vi "Measurement UI.vi"() -> ()   [LabVIEW 2022 SP3, in "Generation_Class D Amplifier_UI.lvlib"]
uses:
  Generation_Class D Amplifier_UI.lvlib
  Generation_Class D Amplifier/generation control.ctl
  shared/controls/digital output level units.ctl
  service/generation/controls/generation status.ctl
  shared/controls/generation type.ctl
  state.ctl
  <vilib>/Utility/miscctls.llb/LVPositionTypeDef.ctl
  <vilib>/Utility/miscctls.llb/LVRowAndColumnTypeDef.ctl
  service/generation/API/AudioGeneration/AudioGeneration.lvclass
  service/generation/controls/generation type.ctl
  service/generation/controls/AudioGenTypeDefs.lvlib
  shared/audio popup ui/Audio Popup UI.lvlib
  shared/controls/audio controls.lvlib
  Generation_Class D Amplifier/Generation_Class D Amplifier.lvlib
  shared/digital serial gen settings/digital audio protocol controls.lvlib
panel:
  out "placeholder":string
  in  "signal parameters":string
  in  "sine wave table":string[][](table)
  in  "DAQmx Physical Channel":tag caption="Analog output channel"
  in  "configure output":bool
  in  "output type":T1 caption="Generation Type"
  in  "master clock channel list":string caption="Master clock channel"
  in  "digital channel list":string caption="Digital audio channel"
  in  "analog output channel":string
  in  "output configuration file":string
  out "status":T2 caption="Status"
  in  "output level units":T3 caption="Output level units"
  in  "generation control":T4=enum."Stop" caption="Action"
  # "Generation"
  # "Harware Resource"
  # "Signals"
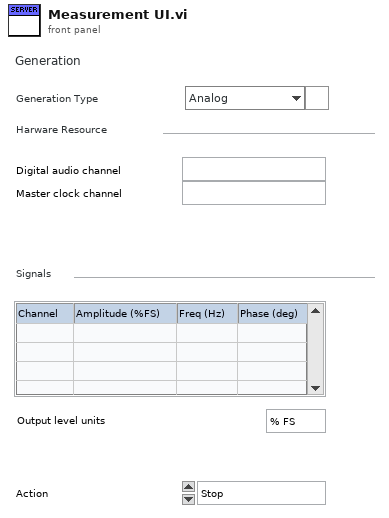
[diagram p1: front panel]
types:
  T1 = typedef "generation type.ctl" = enum32{"Analog", "Digital Serial"}
  T2 = typedef "AudioGenTypeDefs.lvlib/generation status.ctl" = enum16{"Idle", "Committed", "Active"}
  T3 = typedef "audio controls.lvlib/digital output level units.ctl" = enum32{"% FS", "dBFS", "V"}
  T4 = typedef "Generation_Class D Amplifier.lvlib/generation control.ctl" = enum32{"Start", "Stop"}
  T5 = typedef "Generation_Class D Amplifier_UI.lvlib/state.ctl" = cluster{"PostUI event occurred":bool, "digital serial cfg file":path, "analog cfg file":path, "number of channels":u32}
  T6 = typedef "LVPositionTypeDef.ctl" = cluster{"Left":i32, "Top":i32}
  T7 = typedef "LVRowAndColumnTypeDef.ctl" = cluster{"Row":i32, "Column":i32}
  T8 = typedef "AudioGenTypeDefs.lvlib/generation type.ctl" = enum16{"analog", "digital"}
  T9 = cluster{"frequency":dbl, "amplitude":dbl, "phase":dbl}[]
  T10 = typedef "digital serial gen settings.ctl" = cluster{"number of channels":u32, "data justification":T11, "endianness":T12, "channel length":u32, "bit depth":u32, "frame clock rate":dbl, "bit clock edge sync":T13, "master clock rate":dbl, "Logic Level":T14, "frame sync edge for channel 0":T13, "Channel 0 Offset":u32}
  T11 = typedef "PDM Shared.lvlib/PCM Data Justification.ctl" = enum16{"Left Justified", "Right Justified"}
  T12 = typedef "PDM Shared.lvlib/PCM Bit Endianness.ctl" = enum16{"MSB First", "LSB First"}
  T13 = typedef "PDM Shared.lvlib/Digital Edge.ctl" = enum8{"Rising", "Falling"}
  T14 = typedef "PDM Acquisition Class Library.lvlib/DecoderSession.lvclass/Logic Levels.ctl" = enum16{"3.3 V", "1.8 V", "1.2 V"}
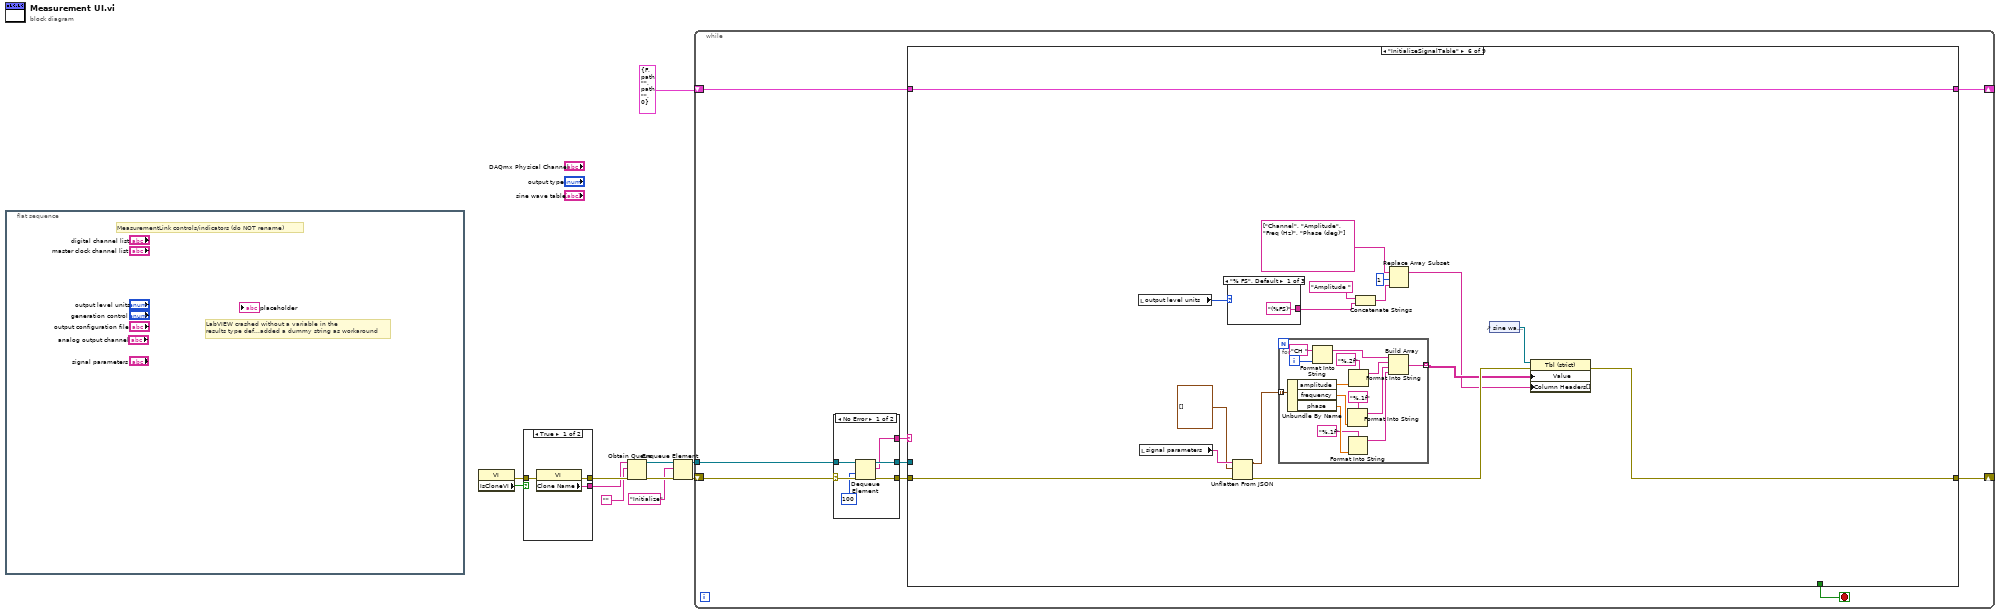
[diagram p0: block diagram]
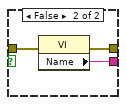
[diagram p2: hidden frame]
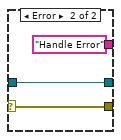
[diagram p3: hidden frame]
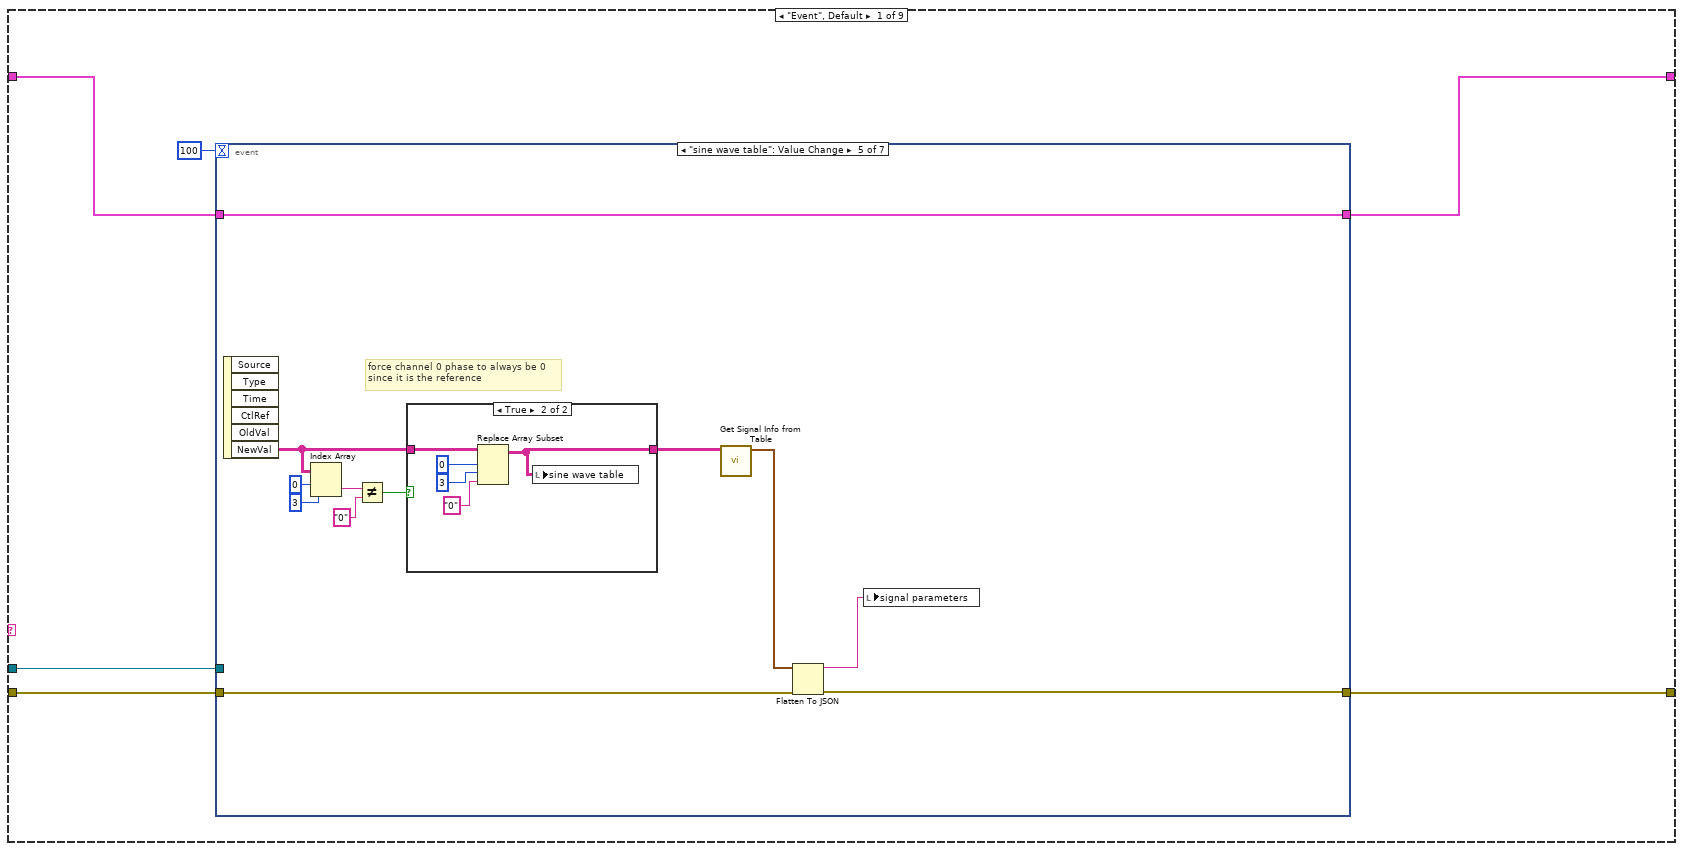
[diagram p4: hidden frame]
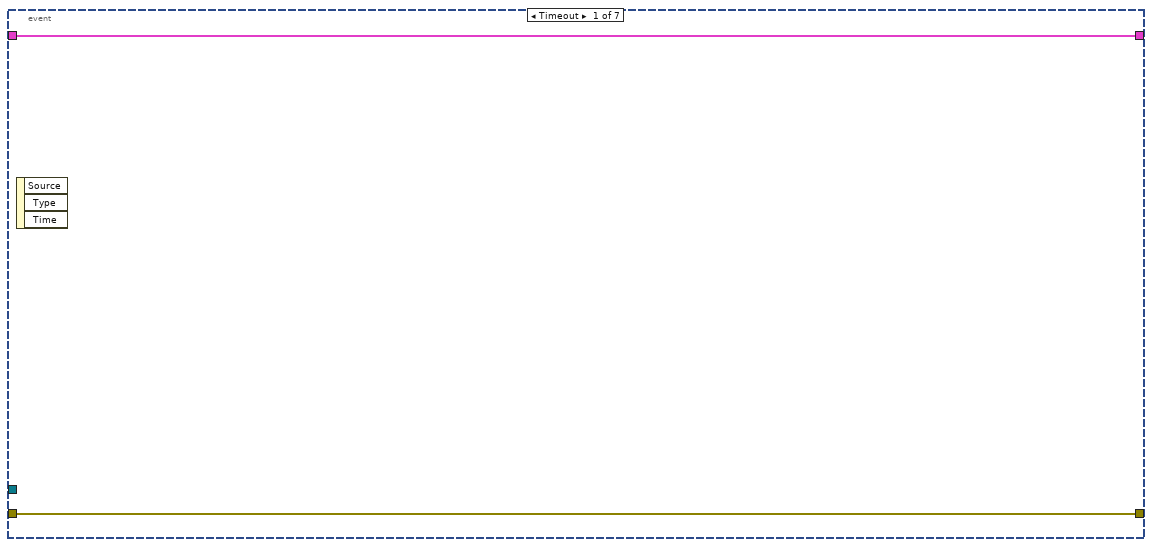
[diagram p5: hidden frame]
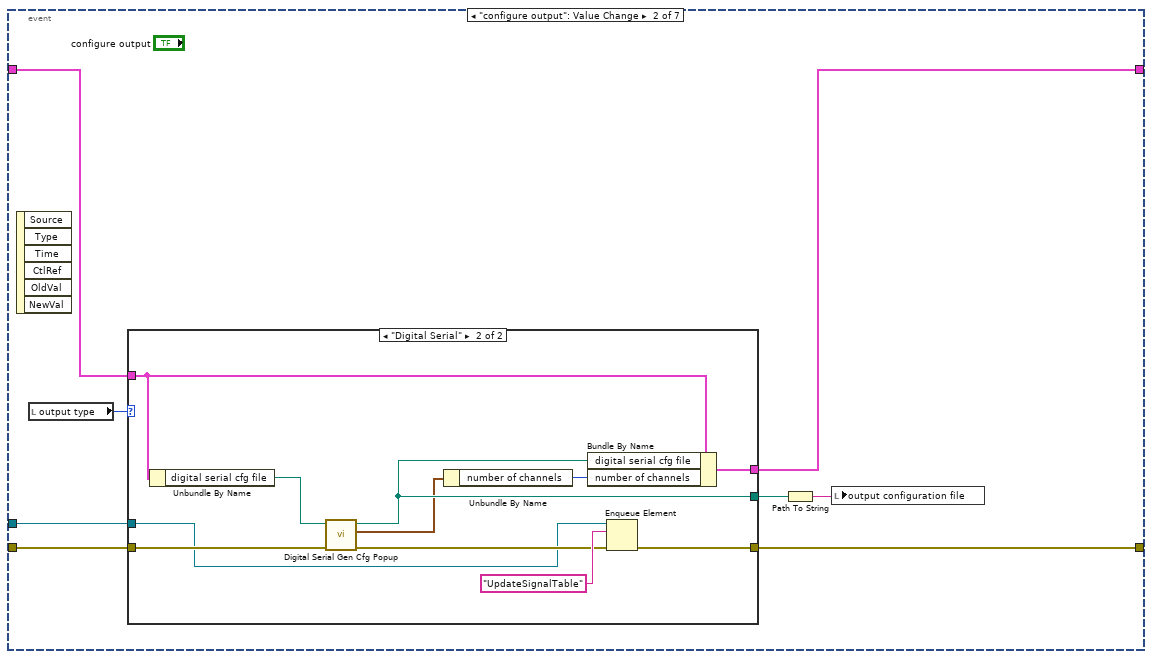
[diagram p6: hidden frame]
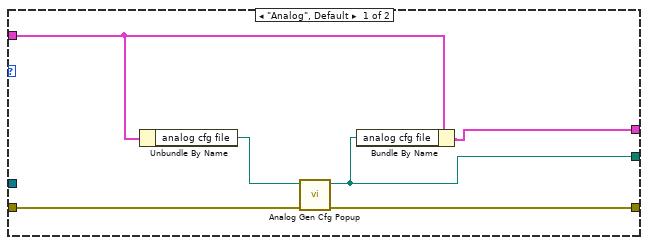
[diagram p7: hidden frame]
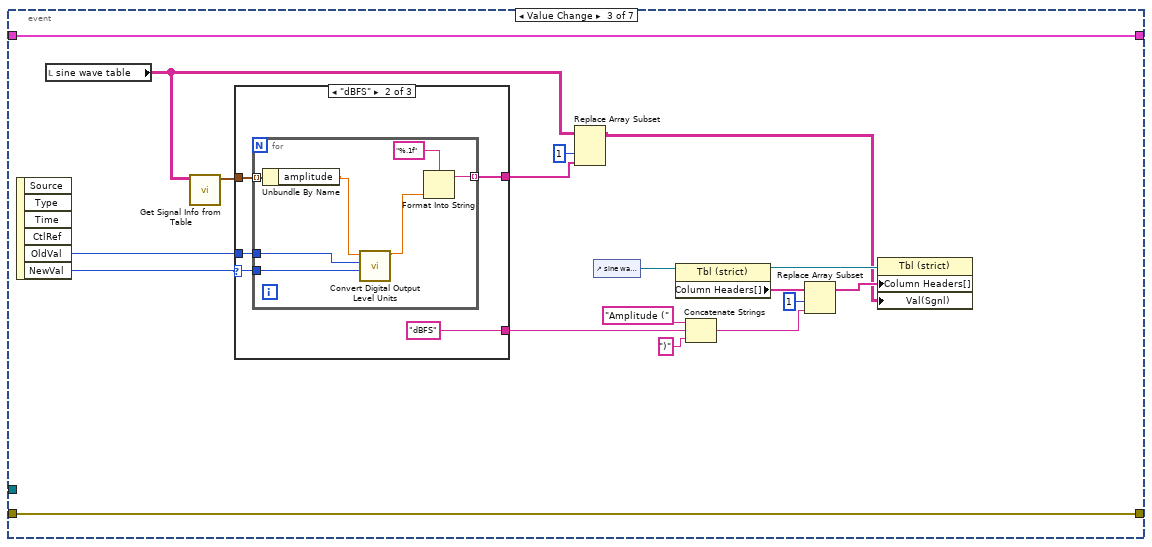
[diagram p8: hidden frame]
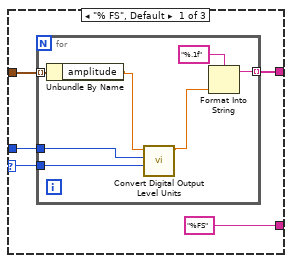
[diagram p9: hidden frame]
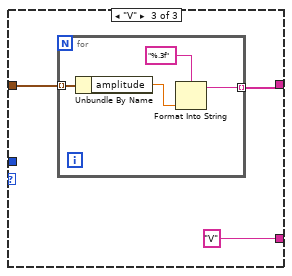
[diagram p10: hidden frame]
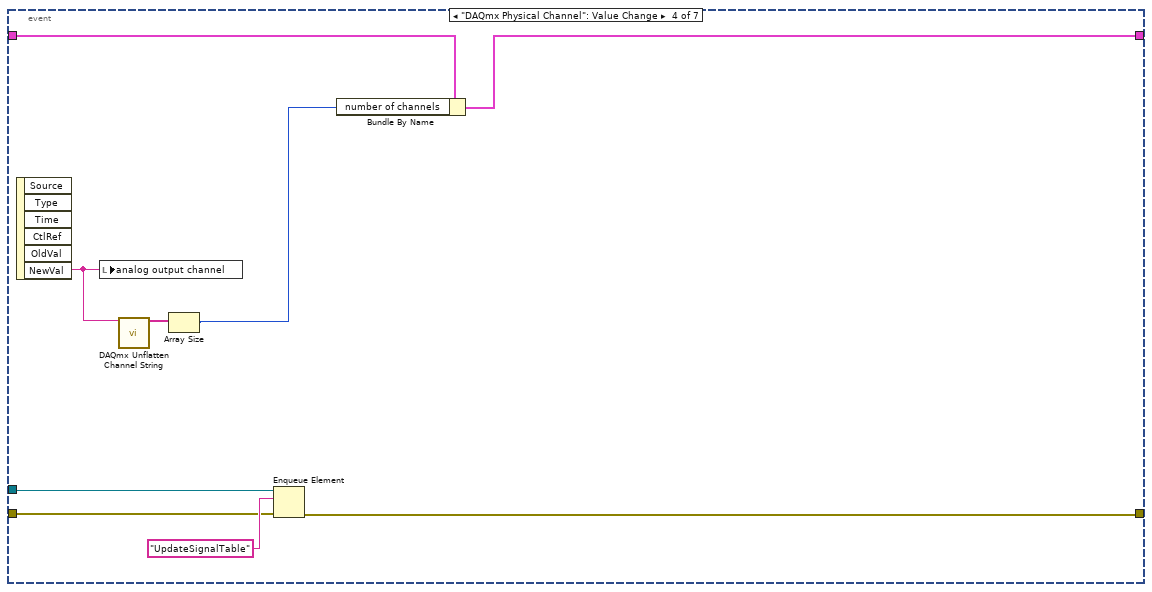
[diagram p11: hidden frame]
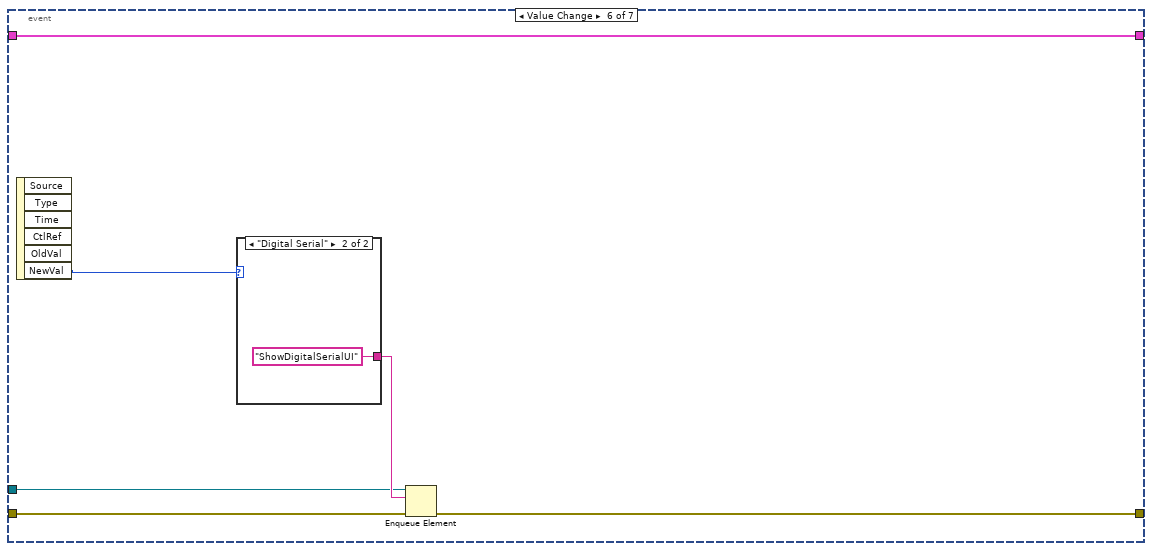
[diagram p13: hidden frame]
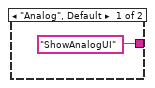
[diagram p14: hidden frame]
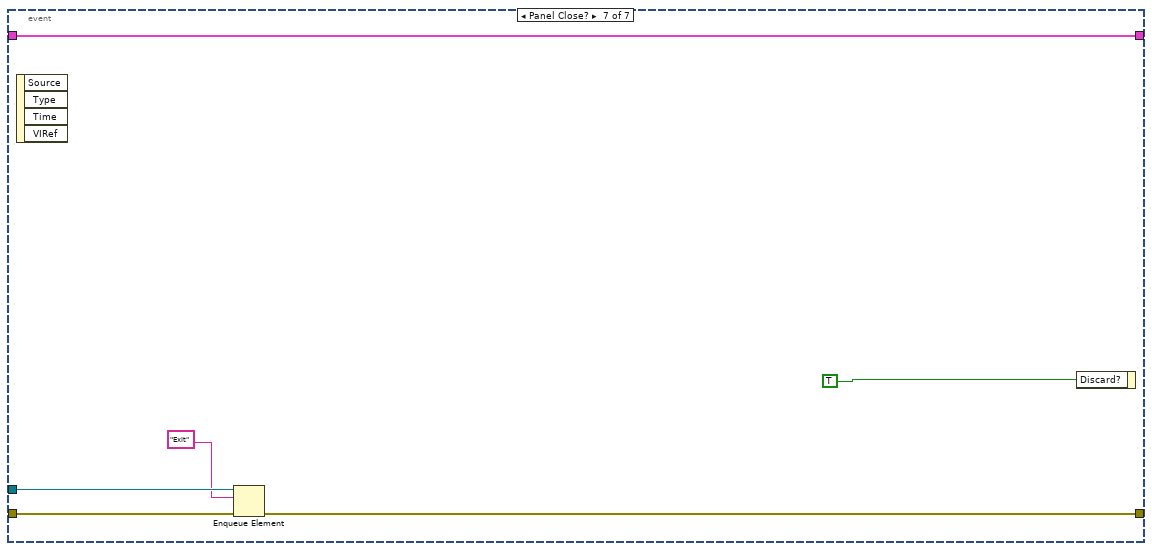
[diagram p15: hidden frame]
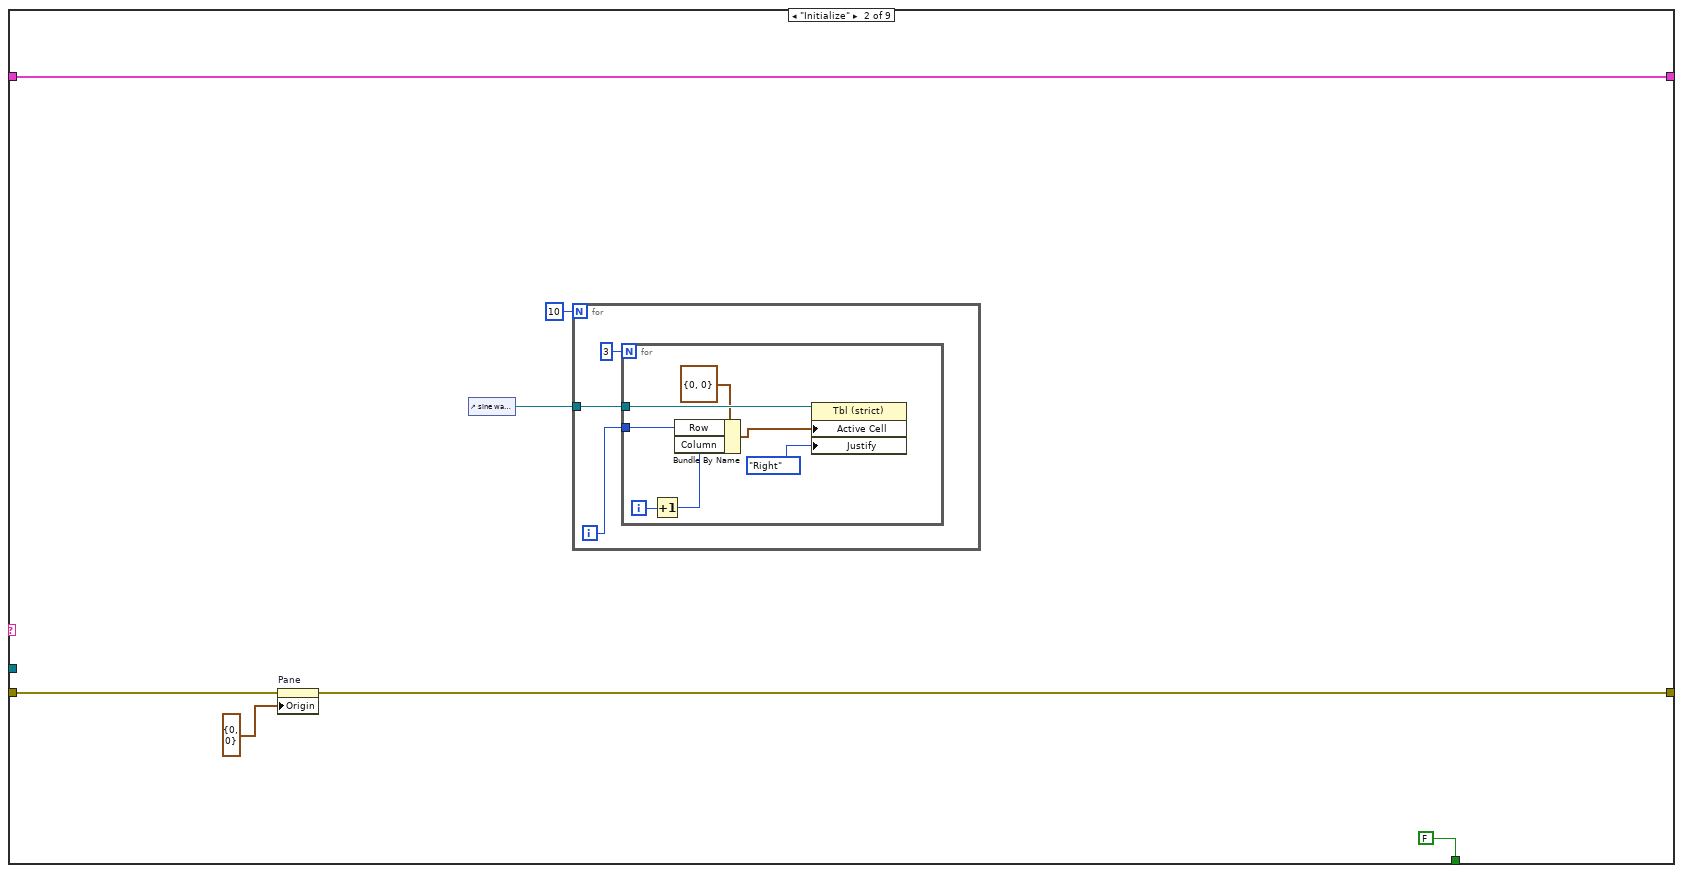
[diagram p16: hidden frame]
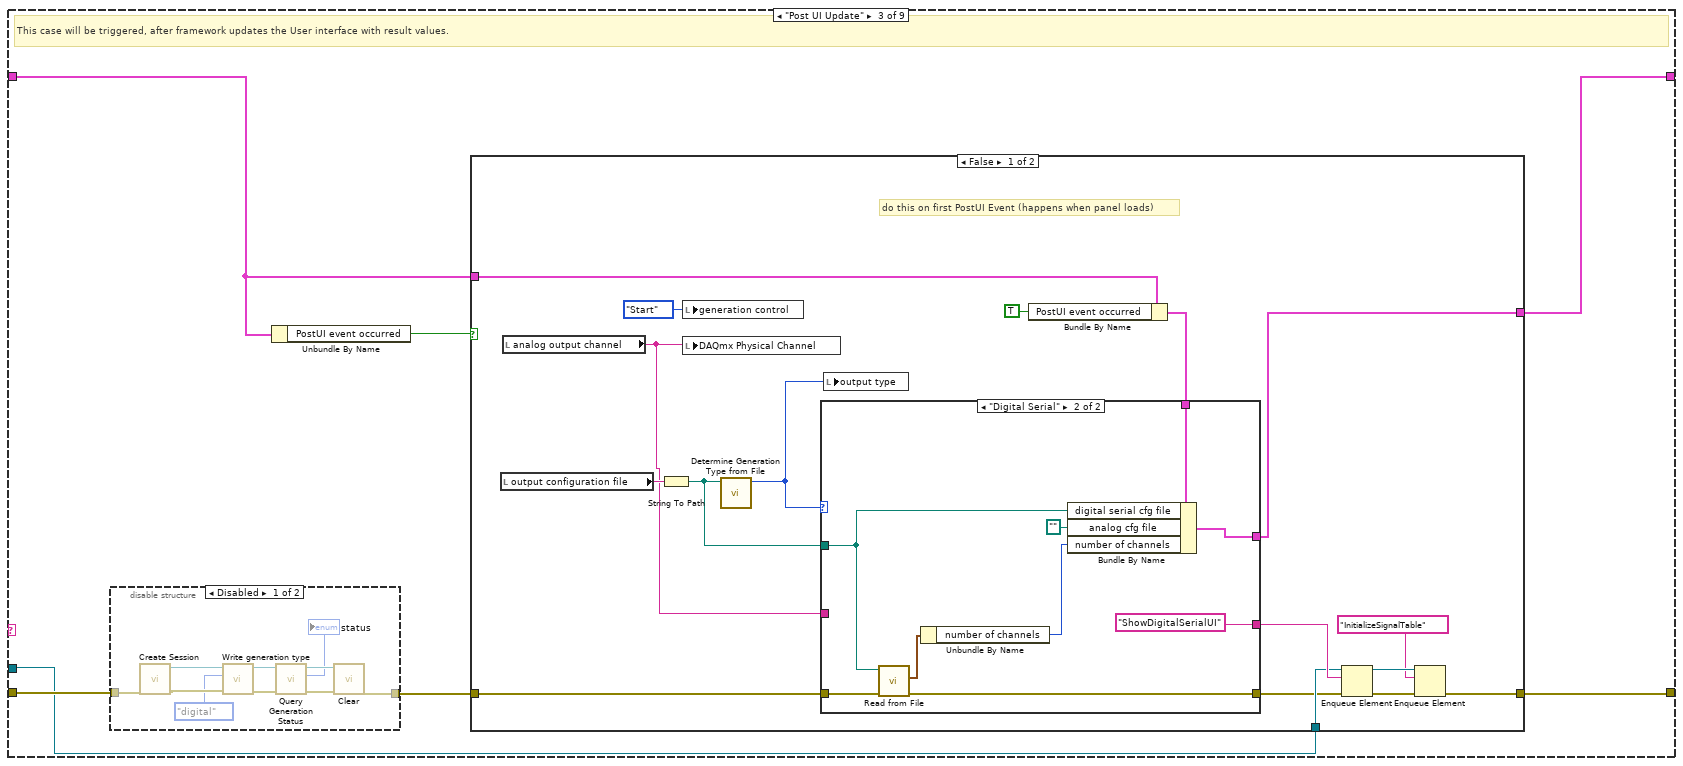
[diagram p17: hidden frame]
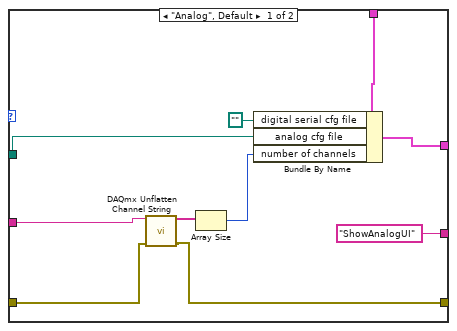
[diagram p19: hidden frame]
diagram:
  n1 = flat-sequence {
    frame #0 {
      # "LabVIEW crashed without a variable in the \nresults type def...added a dummy string as workaround"
      # "MeasurementLink controls/indicators (do NOT rename)"
    }
  }
  n2 = property class="VI"() -> (error out=w2:errorcluster, "IsCloneVI"=w3:bool)  [unwired: 2 in, 1 out]
  n3 = case shown="True" w3 {
    tunnel: [w14 w17] -> w11
    tunnel: [w13 w16] -> w10
    tunnel: w2 -> [w12 w15]
    frame True {
      n4 = property class="VI"(error in=w12) -> (error out=w14:errorcluster, "Clone Name"=w13:string)  [unwired: 1 in, 1 out]
    }
    frame False {
      n5 = property class="VI"(error in=w15) -> (error out=w17:errorcluster, "Name"=w16:string)  [unwired: 1 in, 1 out]
    }
  }
  n6 = Obtain Queue(name (unnamed)=w10, element data type="", error in (no error)=w11) -> (queue out=w7:refnum<queue>, error out=w9:errorcluster)  [unwired: 2 in, 1 out]
  n7 = Enqueue Element(queue=w7, element="Initialize", error in (no error)=w9) -> (queue out=w6:refnum<queue>, error out=w8:errorcluster)  [unwired: 1 in, 1 out]
  n8 = while {
    shift-right: [w21] -> _
    shift-left: w8 -> [w26]
    tunnel: w6 -> [w24]
    shift-right: [w18] -> _
    shift-left: T5 {"PostUI event occurred"=FALSE, "digital serial cfg file"=path "", "analog cfg file"=path "", "number of channels"=0} ("state") -> [w19]
    stop <- w20 stop-if-true
    n9 = case shown="No Error" w26 {
      selector: w26 -> [w32 w35]
      tunnel: [w31 w35] -> w25
      tunnel: w24 -> [w30 w34]
      tunnel: [w29 w34] -> w23
      tunnel: [w28 "Handle Error"] -> w22
      frame No Error {
        n10 = Dequeue Element(queue=w30, timeout in ms (-1)=100, error in (no error)=w32) -> (queue out=w29:refnum<queue>, element=w28:string, error out=w31:errorcluster)  [unwired: 1 out]
      }
      frame Error {
      }
    }
    n11 = case shown="\"InitializeSignalTable\"" w22 {
      tunnel: w25 -> [w40 w164 w182 w238 w254 w275 w302 w331 _]
      tunnel: w23 -> [w38 _ w180 w233 w248 _ _ w329 _]
      tunnel: [w41 w161 w179 w232 w249 w276 w302 w326 errorcluster {"status"=FALSE, "code"=0, "source"=""} ("error out")] -> w21
      tunnel: [_ FALSE _ _ _ _ _ TRUE _] -> w20
      tunnel: w19 -> [w37 w162 w177 w241 w257 w277 w304 w324 w333]
      tunnel: [w36 w162 w176 w240 w256 w277 w304 w324 w333] -> w18
      frame "Event", Default {
        n12 = event shown="[4] \"sine wave table\": Value Change" {
          selector: _ -> [_ _ _ _ _ _ _]
          dyn-events: _ -> [_ _ _ _ _ _ _]
          timeout: 100 -> [_ _ _ _ _ _ _]
          tunnel: [w43 w50 w86 w118 w136 w147 w156] -> w41
          tunnel: w40 -> [w43 w51 w86 w120 w137 w149 w157]
          tunnel: w38 -> [_ w44 _ w119 _ w148 w155]
          tunnel: w37 -> [w42 w46 w83 w123 w138 w145 w153]
          tunnel: [w42 w45 w83 w122 w138 w145 w153] -> w36
          event Timeout {
            n13 = event-data() -> ()  [unwired: 1 in, 3 out]
          }
          event "configure output": Value Change {
            n14 = event-data() -> ()  [unwired: 1 in, 6 out]
            n15 = local read "output type"() -> (w49:T1)
            n16 = case shown="\"Digital Serial\"" w49 {
              tunnel: w51 -> [w57 w68]
              tunnel: [w56 w59] -> w50
              tunnel: [w54 w65] -> w48
              tunnel: w46 -> [w53 w66]
              tunnel: [w52 w64] -> w45
              tunnel: w44 -> [_ w58]
              frame "Analog", Default {
                n17 = Unbundle By Name(w53) -> ("analog cfg file"=w55:path)
                n18 = call "Analog Gen Cfg Popup.vi"("error in (no error)"=w57, "config file in"=w55) -> ("error out"=w56:errorcluster, "config file out"=w54:path)  [unwired: 8 in]
                n19 = Bundle By Name(cluster=w53, "analog cfg file"=w54) -> (w52:T5)
              }
              frame "Digital Serial" {
                n20 = Unbundle By Name(w66) -> ("digital serial cfg file"=w67:path)
                n21 = call "Digital Serial Gen Cfg Popup.vi"("error in (no error)"=w68, "config file in"=w67) -> ("error out"=w60:errorcluster, "digital audio protocol settings"=w63:T10, "config file out"=w65:path)  [unwired: 7 in]
                n22 = Unbundle By Name(w63) -> ("number of channels"=w62:u32)
                n23 = Bundle By Name(cluster=w66, "digital serial cfg file"=w65, "number of channels"=w62) -> (w64:T5)
                n24 = Enqueue Element(queue=w58, element="UpdateSignalTable", error in (no error)=w60) -> (error out=w59:errorcluster)  [unwired: 1 in, 2 out]
              }
            }
            n25 = Path To String(path=w48) -> (string=w47:string)
            n26 = local write "output configuration file"(w47) -> ()
          }
          event Value Change {
            n27 = event-data() -> ("OldVal"=w85:T3, "NewVal"=w84:T3)  [unwired: 1 in, 4 out]
            n28 = local read "sine wave table"() -> (w72:string[][])
            n29 = call "Get Signal Info from Table.vi"("signal table"=w72) -> ("signal parameters"=w73:T9)  [unwired: 10 in]
            n30 = case shown="\"dBFS\"" w84 {
              selector: w84 -> [w90 w100 _]
              tunnel: w85 -> [w91 w101 _]
              tunnel: w73 -> [w88 w102 w112]
              tunnel: ["%FS" ("string") "dBFS" ("string") "V" ("string")] -> w74
              tunnel: [w87 w99 w111] -> w70
              frame "% FS", Default {
                n31 = for {
                  tunnel: w91 -> [w98]
                  tunnel: w90 -> [w97]
                  tunnel: w88 -> [w96] mode=indexing
                  tunnel: [w93] -> w87 mode=indexing
                  n32 = Unbundle By Name(w96) -> ("amplitude"=w95:dbl)
                  n33 = call "Convert Digital Output Level Units.vi"("new output level units"=w97, "previous output level units"=w98, "previous output level"=w95) -> ("new output level"=w94:dbl)  [unwired: 8 in]
                  n34 = Format Into String(format string="%.1f", w94) -> (resulting string=w93:string)  [unwired: 2 in, 1 out]
                }
              }
              frame "dBFS" {
                n35 = for {
                  tunnel: w101 -> [w110]
                  tunnel: w100 -> [w109]
                  tunnel: w102 -> [w108] mode=indexing
                  tunnel: [w105] -> w99 mode=indexing
                  n36 = Unbundle By Name(w108) -> ("amplitude"=w107:dbl)
                  n37 = call "Convert Digital Output Level Units.vi"("new output level units"=w109, "previous output level units"=w110, "previous output level"=w107) -> ("new output level"=w106:dbl)  [unwired: 8 in]
                  n38 = Format Into String(format string="%.1f", w106) -> (resulting string=w105:string)  [unwired: 2 in, 1 out]
                }
              }
              frame "V" {
                n39 = for {
                  tunnel: w112 -> [w117] mode=indexing
                  tunnel: [w115] -> w111 mode=indexing
                  n40 = Unbundle By Name(w117) -> ("amplitude"=w116:dbl)
                  n41 = Format Into String(format string="%.3f", w116) -> (resulting string=w115:string)  [unwired: 2 in, 1 out]
                }
              }
            }
            n42 = Replace Array Subset(array=w72, new element=w70, index (col)=1 ("disabled index (col)")) -> (w69:string[][])  [unwired: 1 in]
            n43 = control-ref of="sine wave table"() -> (w82:refnum<vi>)
            n44 = property class="Tbl (strict)"(reference=w82) -> (reference out=w81:refnum<vi>, "Column Headers[]"=w80:string[])  [unwired: 1 in, 1 out]
            n45 = Concatenate Strings("Amplitude (" ("string"), w74, ")" ("string")) -> (w75:string)
            n46 = Replace Array Subset(array=w80, new element=w75, index=1) -> (w78:string[])
            n47 = property class="Tbl (strict)"(reference=w81, "Column Headers[]"=w78, "Val(Sgnl)"=w69) -> ()  [unwired: 1 in, 2 out]
          }
          event "DAQmx Physical Channel": Value Change {
            n48 = event-data() -> ("NewVal"=w126:tag)  [unwired: 1 in, 5 out]
            n49 = local write "analog output channel"(w126) -> ()
            n50 = call <vilib>:"DAQmx Unflatten Channel String.vi"("names in"=w126) -> ("names out"=w125:string[])  [unwired: 13 in, 1 out]
            n51 = Array Size(array=w125) -> (size(s)=w124:i32)
            n52 = Enqueue Element(queue=w119, element="UpdateSignalTable", error in (no error)=w120) -> (error out=w118:errorcluster)  [unwired: 1 in, 2 out]
            n53 = Bundle By Name(cluster=w123, "number of channels"=w124) -> (w122:T5)
          }
          event "sine wave table": Value Change {
            # "force channel 0 phase to always be 0\nsince it is the reference"
            n54 = event-data() -> ("NewVal"=w129:string[][])  [unwired: 1 in, 5 out]
            n55 = Index Array(array=w129, index (row)=0, index (col)=3 ("disabled index (col)")) -> (element=w132:string)
            n56 = Not Equal?(x=w132, y="0") -> (x != y?=w130:bool)
            n57 = case shown="True" w130 {
              tunnel: w129 -> [w139 w144]
              tunnel: [w139 w140] -> w128
              frame False {
              }
              frame True {
                n58 = Replace Array Subset(array=w144, new element="0" ("new element/subarray"), index (row)=0, index (col)=3 ("disabled index (col)")) -> (w140:string[][])
                n59 = local write "sine wave table"(w140) -> ()
              }
            }
            n60 = call "Get Signal Info from Table.vi"("signal table"=w128) -> ("signal parameters"=w127:T9)  [unwired: 10 in]
            n61 = Flatten To JSON(anything=w127, error in (no error)=w137) -> (JSON string=w135:string, 11:w136:errorcluster)  [unwired: 1 in]
            n62 = local write "signal parameters"(w135) -> ()
          }
          event Value Change {
            n63 = event-data() -> ("NewVal"=w146:T1)  [unwired: 1 in, 5 out]
            n64 = case shown="\"Digital Serial\"" w146 {
              tunnel: ["ShowAnalogUI" ("element") "ShowDigitalSerialUI" ("element")] -> w150
              frame "Analog", Default {
              }
              frame "Digital Serial" {
              }
            }
            n65 = Enqueue Element(queue=w148, element=w150, error in (no error)=w149) -> (error out=w147:errorcluster)  [unwired: 1 in, 2 out]
          }
          event Panel Close? {
            n66 = event-data() -> ()  [unwired: 1 in, 4 out]
            n67 = Enqueue Element(queue=w155, element="Exit", error in (no error)=w157) -> (error out=w156:errorcluster)  [unwired: 1 in, 2 out]
            n68 = event-data("Discard?"=TRUE) -> ()  [unwired: 1 in, 1 out]
          }
        }
      }
      frame "Initialize" {
        n69 = property on="Pane" class="Pane"(error in=w164, "Origin"=T6 {"Left"=0, "Top"=0} ("Position")) -> (error out=w161:errorcluster)  [unwired: 1 in, 1 out]
        n70 = control-ref of="sine wave table"() -> (w160:refnum<vi>)
        n71 = for {
          N: 10 -> [_]
          tunnel: w160 -> [w168]
          i -> [w166]
          n72 = for {
            N: 3 -> [_]
            tunnel: w168 -> [w175]
            tunnel: w166 -> [w169]
            i -> [w171]
            n73 = Increment(x=w171) -> (x+1=w170:i32)
            n74 = Bundle By Name(cluster=T7 {"Row"=0, "Column"=0} ("Active Cell:Active Cell"), "Row"=w169, "Column"=w170) -> (w173:T7)
            n75 = property class="Tbl (strict)"(reference=w175, "Active Cell"=w173, "Justify"=enum16{"Left", "Center", "Right"}."Right" ("Active Cell:Cell Justification")) -> ()  [unwired: 1 in, 2 out]
          }
        }
      }
      frame "Post UI Update" {
        # "This case will be triggered, after framework updates the User interface with result values."
        n76 = disable-structure shown="Disabled" {
          disable-tunnel: w182 -> [w192 w193]
          disable-tunnel: [w183 w193] -> w181
          frame Disabled {
            n77 = call "Create Session.vi"("error in (no error)"=w192) -> ("error out"=w190:errorcluster, "session out"=w191:refnum<class "AudioGeneration.lvclass">)  [unwired: 9 in]
            n78 = call-dynamic "Write generation type.vi"("error in (no error)"=w190, "generation type"=generation_type."digital", "AudioGeneration in"=w191) -> ("error out"=w188:errorcluster, "AudioGeneration out"=w189:refnum<class "AudioGeneration.lvclass">)  [unwired: 7 in]
            n79 = call "Query Generation Status.vi"("error in (no error)"=w188, "AudioGeneration in"=w189) -> ("error out"=w187:errorcluster, "status"=→"status":T2, "AudioGeneration out"=w186:refnum<class "AudioGeneration.lvclass">)  [unwired: 5 in, 2 out]
            n80 = call "Clear.vi"("error in (no error)"=w187, "AudioGeneration in"=w186) -> ("error out"=w183:errorcluster)  [unwired: 9 in]
          }
          frame Enabled {
          }
        }
        n81 = Unbundle By Name(w177) -> ("PostUI event occurred"=w178:bool)
        n82 = case shown="False" w178 {
          tunnel: w181 -> [w199 w231]
          tunnel: w180 -> [w207 _]
          tunnel: [w196 w231] -> w179
          tunnel: w177 -> [w206 w230]
          tunnel: [w203 w230] -> w176
          frame False {
            # "do this on first PostUI Event (happens when panel loads)"
            n83 = local read "output configuration file"() -> (w210:string)
            n84 = local read "analog output channel"() -> (w200:string)
            n85 = String To Path(string=w210) -> (path=w202:path)
            n86 = local write "generation control"(generation_control."Start" ("generation control")) -> ()
            n87 = local write "DAQmx Physical Channel"(w200) -> ()
            n88 = call "Determine Generation Type from File.vi"("cfg file"=w202) -> ("output type"=w208:T1)  [unwired: 9 in, 1 out]
            n89 = local write "output type"(w208) -> ()
            n90 = Bundle By Name(cluster=w206, "PostUI event occurred"=TRUE) -> (w204:T5)
            n91 = case shown="\"Digital Serial\"" w208 {
              tunnel: ["ShowAnalogUI" ("element") "ShowDigitalSerialUI" ("element")] -> w209
              tunnel: w204 -> [w219 w228]
              tunnel: [w218 w227] -> w203
              tunnel: w202 -> [w216 w223]
              tunnel: w200 -> [w214 _]
              tunnel: w199 -> [w212 w225]
              tunnel: [w211 w224] -> w198
              frame "Analog", Default {
                n92 = call <vilib>:"DAQmx Unflatten Channel String.vi"("names in"=w214, "error in"=w212) -> ("names out"=w215:string[], "error out"=w211:errorcluster)  [unwired: 12 in]
                n93 = Array Size(array=w215) -> (size(s)=w213:i32)
                n94 = Bundle By Name(cluster=w219, "digital serial cfg file"=path "", "analog cfg file"=w216, "number of channels"=w213) -> (w218:T5)
              }
              frame "Digital Serial" {
                n95 = call "Read from File.vi"("error in (no error)"=w225, "file path"=w223) -> ("error out"=w224:errorcluster, "digital audio protocol settings"=w222:T10)  [unwired: 7 in, 1 out]
                n96 = Unbundle By Name(w222) -> ("number of channels"=w221:u32)
                n97 = Bundle By Name(cluster=w228, "digital serial cfg file"=w223, "analog cfg file"=path "", "number of channels"=w221) -> (w227:T5)
              }
            }
            n98 = Enqueue Element(queue=w207, element=w209, error in (no error)=w198) -> (queue out=w195:refnum<queue>, error out=w197:errorcluster)  [unwired: 1 in, 1 out]
            n99 = Enqueue Element(queue=w195, element="InitializeSignalTable", error in (no error)=w197) -> (error out=w196:errorcluster)  [unwired: 1 in, 2 out]
          }
          frame True {
          }
        }
      }
      frame "ShowAnalogUI" {
        w245 = T3[] [enum."% FS", enum."dBFS"] items=["% FS", "dBFS", "V"]
        w244 = FALSE ("Visible")
        n100 = Unbundle By Name(w241) -> ("analog cfg file"=w243:path)
        n101 = local read "analog output channel"() -> (w236:string)
        n102 = Path To String(path=w243) -> (string=w242:string)
        n103 = local write "output configuration file"(w242) -> ()
        n104 = call <vilib>:"DAQmx Unflatten Channel String.vi"("names in"=w236, "error in"=w238) -> ("names out"=w239:string[], "error out"=w234:errorcluster)  [unwired: 12 in]
        n105 = Array Size(array=w239) -> (size(s)=w237:i32)
        n106 = Bundle By Name(cluster=w241, "number of channels"=w237) -> (w240:T5)
        n107 = Enqueue Element(queue=w233, element="UpdateSignalTable", error in (no error)=w234) -> (error out=w232:errorcluster)  [unwired: 1 in, 2 out]
        n108 = property on="master clock channel list" class="Str"("Visible"=w244) -> ()  [unwired: 2 in, 2 out]
        n109 = property on="digital channel list" class="Str"("Visible"=w244) -> ()  [unwired: 2 in, 2 out]
        n110 = property on="DAQmx Physical Channel" class="DAQmxName"("Visible"=TRUE) -> ()  [unwired: 2 in, 2 out]
        n111 = property on="output level units" class="Enum (strict)"("Disabled Items []"=w245, "Value"=digital_output_level_units."V" ("output level units")) -> ()  [unwired: 2 in, 2 out]
      }
      frame "ShowDigitalSerialUI" {
        w261 = T3[] [enum."V"] items=["% FS", "dBFS", "V"]
        w259 = TRUE ("Visible")
        n112 = Unbundle By Name(w257) -> ("digital serial cfg file"=w252:path)
        n113 = Path To String(path=w252) -> (string=w258:string)
        n114 = call "Read from File.vi"("error in (no error)"=w254, "file path"=w252) -> ("error out"=w250:errorcluster, "digital audio protocol settings"=w255:T10)  [unwired: 7 in, 1 out]
        n115 = local write "output configuration file"(w258) -> ()
        n116 = Unbundle By Name(w255) -> ("number of channels"=w253:u32)
        n117 = Bundle By Name(cluster=w257, "number of channels"=w253) -> (w256:T5)
        n118 = Enqueue Element(queue=w248, element="UpdateSignalTable", error in (no error)=w250) -> (error out=w249:errorcluster)  [unwired: 1 in, 2 out]
        n119 = property on="master clock channel list" class="Str"("Visible"=w259) -> ()  [unwired: 2 in, 2 out]
        n120 = property on="output level units" class="Enum (strict)"("Disabled Items []"=w261, "Val(Sgnl)"=digital_output_level_units."% FS" ("output level units")) -> ()  [unwired: 2 in, 2 out]
        n121 = property on="digital channel list" class="Str"("Visible"=w259) -> ()  [unwired: 2 in, 2 out]
        n122 = property on="DAQmx Physical Channel" class="DAQmxName"("Visible"=FALSE) -> ()  [unwired: 2 in, 2 out]
      }
      frame "InitializeSignalTable" {
        n123 = local read "output level units"() -> (w266:T3)
        n124 = local read "signal parameters"() -> (w273:string)
        n125 = case shown="\"% FS\", Default" w266 {
          tunnel: ["(%FS)" ("string") "(dBFS)" ("string") "(V)" ("string")] -> w263
          frame "% FS", Default {
          }
          frame "dBFS" {
          }
          frame "V" {
          }
        }
        n126 = Unflatten From JSON(JSON string=w273, type and defaults=T9 [], error in (no error)=w275) -> (value=w271:T9, error out=w274:errorcluster)  [unwired: 4 in]
        n127 = for {
          tunnel: [w292] -> w270 mode=indexing
          tunnel: w271 -> [w291] mode=indexing
          i -> [w294]
          n128 = Unbundle By Name(w291) -> ("amplitude"=w290:dbl, "frequency"=w288:dbl, "phase"=w286:dbl)
          n129 = Format Into String(initial string="CH ", w294) -> (resulting string=w293:string)  [unwired: 2 in, 1 out]
          n130 = Format Into String(format string="%.1f", w288) -> (resulting string=w287:string)  [unwired: 2 in, 1 out]
          n131 = Format Into String(format string="%.1f", w286) -> (resulting string=w285:string)  [unwired: 2 in, 1 out]
          n132 = Format Into String(format string="%.2f", w290) -> (resulting string=w289:string)  [unwired: 2 in, 1 out]
          n133 = Build Array(w293, w289, w287, w285) -> (w292:string[])
        }
        n134 = Concatenate Strings("Amplitude " ("string"), w263) -> (w265:string)
        n135 = Replace Array Subset(array=string[] ["Channel", "Amplitude", "Freq (Hz)", "Phase (deg)"] ("Column Header Strings[]"), new element=w265, index=1) -> (w268:string[])
        n136 = control-ref of="sine wave table"() -> (w278:refnum<vi>)
        n137 = property class="Tbl (strict)"(reference=w278, error in=w274, "Value"=w270, "Column Headers[]"=w268) -> (error out=w276:errorcluster)  [unwired: 1 out]
      }
      frame "UpdateSignalTable" {
        n138 = local read "sine wave table"() -> (w298:string[][])
        n139 = Unbundle By Name(w304) -> ("number of channels"=w300:u32)
        n140 = Array Size(array=w298) -> (size(s)=w303:i32[])
        n141 = To Long Integer(number=w300) -> (32bit integer=w299:i32)
        n142 = Index Array(array=w303) -> (element=w297:i32)  [unwired: 1 in]
        n143 = Subtract(x=w297, y=w299) -> (x-y=w301:i32)
        n144 = case shown="..-1" w301 {
          selector: w301 -> [_ w307 w314]
          tunnel: w298 -> [w305 w308 w311]
          tunnel: w297 -> [_ _ w312]
          tunnel: [w305 w306 w309] -> w296
          frame 0, Default {
            # "same number of channels;\ndon't change anything"
          }
          frame 1.. {
            # "need to remove channels"
            n145 = Delete From Array(array=w308, length=w307) -> (array with subset deleted=w306:string[][])  [unwired: 2 in, 1 out]
          }
          frame ..-1 {
            # "need to add channels"
            n146 = Absolute Value(x=w314) -> (abs(x)=w313:i32)
            n147 = for {
              N: w313 -> [_]
              tunnel: w312 -> [w320]
              tunnel: [w315] -> w310 mode=indexing
              i -> [w321]
              n148 = Add(x=w320, y=w321) -> (x+y=w322:i32)
              n149 = Format Into String(initial string="CH ", w322) -> (resulting string=w319:string)  [unwired: 2 in, 1 out]
              n150 = Build Array(w319, "1" ("element"), "1000" ("element"), "0" ("element")) -> (w315:string[])
            }
            n151 = Build Array (concatenate)(w311, w310) -> (w309:string[][])
          }
        }
        n152 = property on="sine wave table" class="Tbl (strict)"("Val(Sgnl)"=w296) -> ()  [unwired: 2 in, 2 out]
      }
      frame "Exit" {
        # "This case is triggered to close the User Interface from framework"
        n153 = Flush Queue(queue=w329, error in (no error)=w331) -> (queue out=w328:refnum<queue>, error out=w327:errorcluster)  [unwired: 1 out]
        n154 = Release Queue(queue=w328, force destroy? (F)=TRUE, error in (no error)=w327) -> (error out=w326:errorcluster)  [unwired: 2 out]
      }
      frame "Handle Error" {
      }
    }
  }
